vi "analiza_lvm.vi"() -> ()   [LabVIEW 2014]
uses:
  <vilib>/express/express analysis/Spectral/Block/exnSpectralBlock spectral measurements peak poly.vi
  <vilib>/express/express analysis/Spectral/Block/exnSpectralBlock spectral measurements peak DDT.vi
  <vilib>/express/express analysis/Spectral/XNode/ExpressSpectralMeasurementsBlockNode.xnode
panel:
  out "Dominantna frekvencija":dbl
  out "Peak_to_Peak":dbl
  out "RMS":dbl
  out "Vibracije frekvencijski domen":dynamicdata(graph)
  out "Vibracije vremenski domen":dynamicdata(graph) caption="Signals"
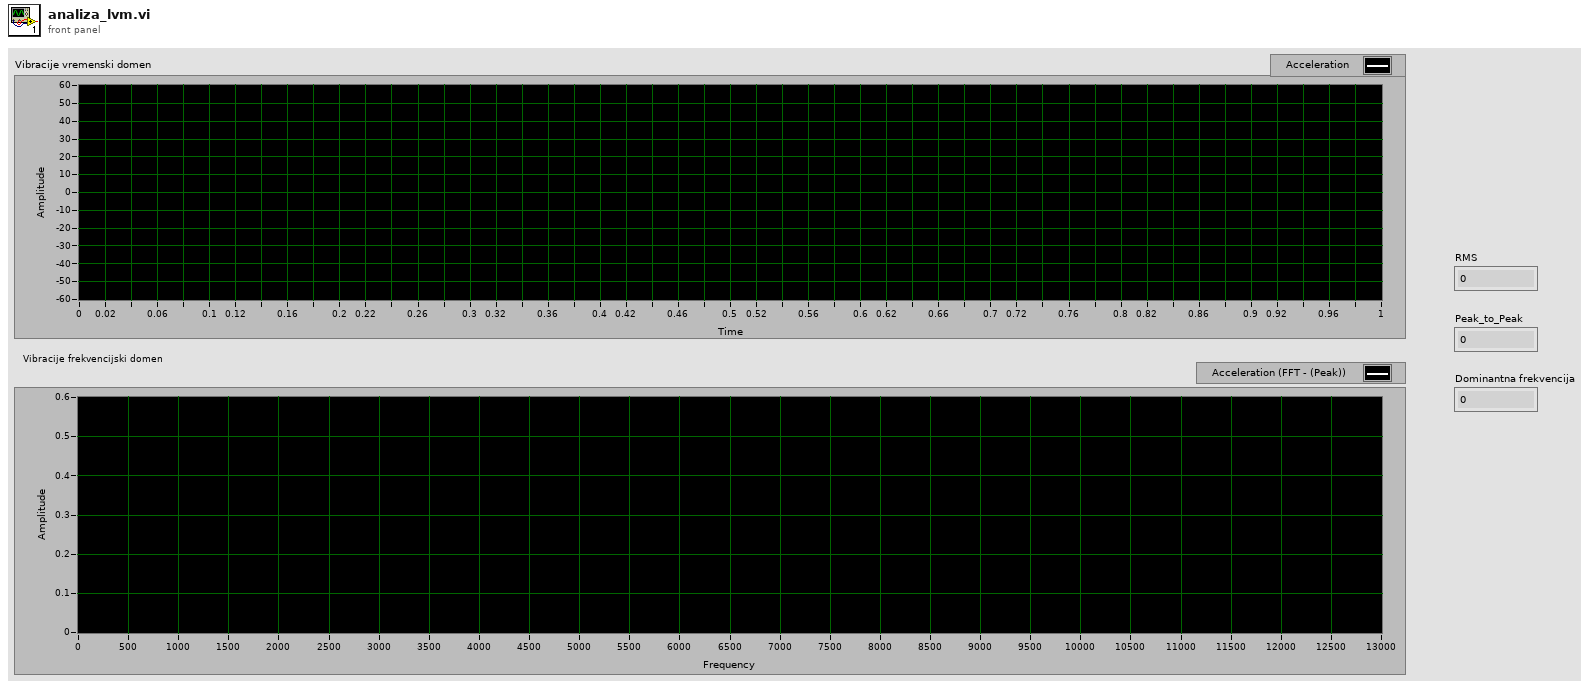
[diagram p1: front panel]
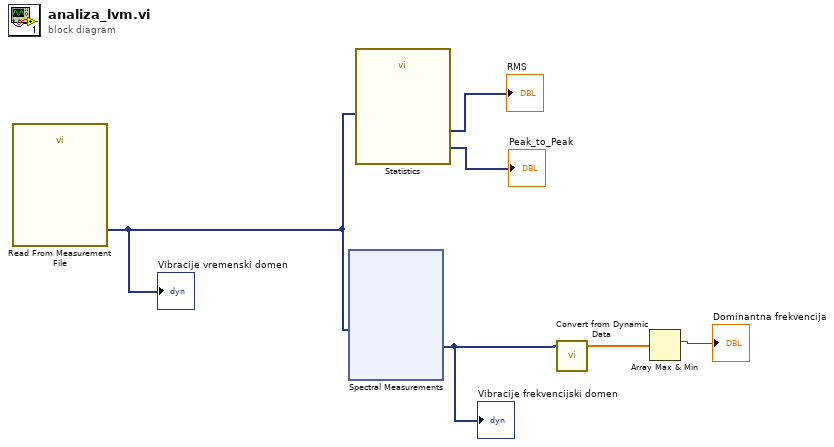
[diagram p0: block diagram]
diagram:
  n1 = call "Read From Measurement File"() -> ("Signals"=w6:dynamicdata)  [unwired: 6 in, 5 out]
  "Vibracije vremenski domen" <- w6
  n2 = xnode "Spectral Measurements"("Signals"=w6) -> ("FFT - (Peak)"=w2:dynamicdata)  [unwired: 1 in, 2 out]
  "Vibracije frekvencijski domen" <- w2
  n3 = call "Statistics"("Signals"=w6) -> ("RMS"=→"RMS":dynamicdata, "Range"=→"Peak_to_Peak":dynamicdata)  [unwired: 24 in, 1 out]
  n4 = call "Convert from Dynamic Data"("Dynamic Data Type"=w2) -> ("Array"=w3:dbl[])  [unwired: 3 in]
  n5 = Array Max & Min(array=w3) -> (max index (indices)=→"Dominantna frekvencija":i32)  [unwired: 3 out]
